vi "measure BT Frequency Separation Step1.vi"(8 "error in (no error)":errorcluster, 11 "SA Measurement in":refnum<class "SA Measurement.lvclass">) -> (0 "error out":errorcluster, 3 "SA Measurement out":refnum<class "SA Measurement.lvclass">)   [LabVIEW 2023, in "Spectrum Analyzer.lvlib" / "SA Measurement.lvclass"]
uses:
  SA Measurement.lvclass
  SA Measurement.lvclass/SA Measurement.ctl
  TYPE DEFINITION/Keysight 9020A/TYPE Measurement Preset.ctl
  Spectrum Analyzer.lvlib
  TYPE DEFINITION/TYPE RBW and VBW Select.ctl
  Interface_Spectrum/Interface_Spectrum.lvclass
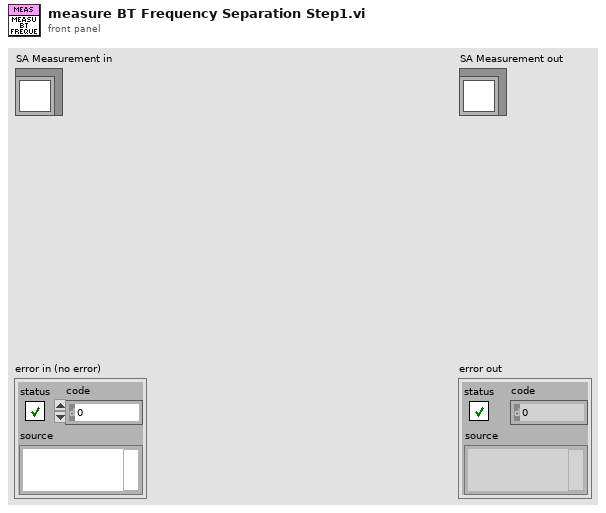
[diagram p1: front panel]
types:
  T1 = typedef "Spectrum Analyzer.lvlib/TYPE RBW and VBW Select.ctl" = enum16{"Res BW", "Video BW"}
  T2 = typedef "Spectrum Analyzer.lvlib/TYPE Measurement Preset.ctl" = enum16{"Sweep SA Mode", "Channel Power", "Occupied BW", "ACP", "Spurious Emission", "Spurious Emission Mask", "Burst Power (Transmit Power)"}
  T3 = typedef "Spectrum Analyzer.lvlib/TYPE Reference Level and Atten Param.ctl" = cluster{"Reference Level":dbl, "Atten":i32, "Atten Auto?":bool, "Reference Level Offset":dbl}
  T4 = typedef "Spectrum Analyzer.lvlib/TYPE Display Trace Mode Select.ctl" = enum16{"Clear Write", "Max Hold", "Min Hold", "Average", "View"}
  T5 = typedef "Spectrum Analyzer.lvlib/TYPE Detect Mode Select.ctl" = enum16{"Det Auto (Normal)", "Auto Peak", "Positive Peak", "Negative Peak", "Sample", "RMS", "Average", "Quasipeak", "CISPR Average", "RMS Average"}
  T6 = cluster{"Trace Mode":T4, "Detector Type":T5, "Detect Auto?":bool}[]
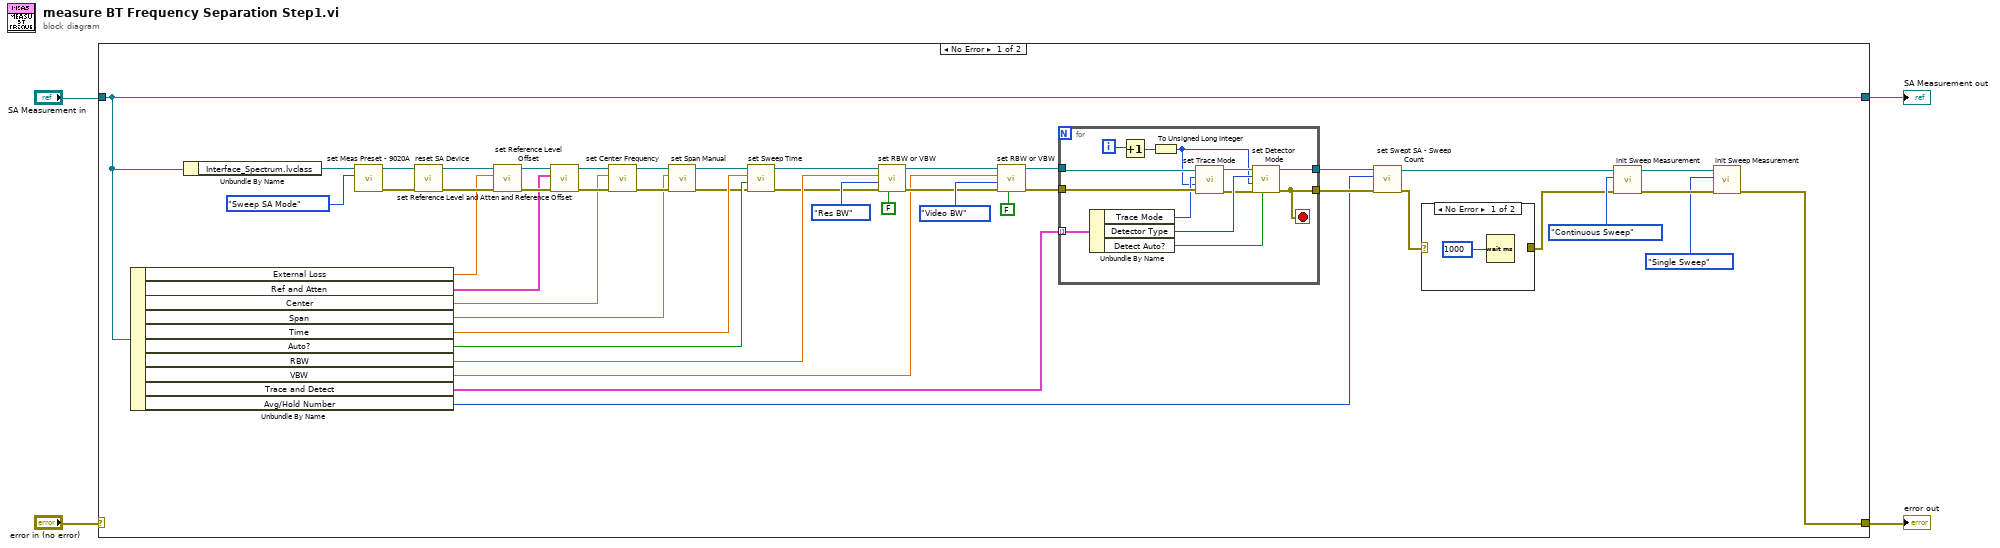
[diagram p0: block diagram]
diagram:
  n1 = case shown="No Error" "error in (no error)" {
    selector: "error in (no error)" -> [_ w66]
    tunnel: [w5 w66] -> w1
    tunnel: [w19 w65] -> w2
    tunnel: "SA Measurement in" -> [w19 w65]
    frame No Error {
      n2 = Unbundle By Name(w19) -> ("External Loss"=w41:dbl, "Ref and Atten"=w40:T3, "Center"=w16:dbl, "Span"=w13:dbl, "Time"=w25:dbl, "Auto?"=w24:bool, "RBW"=w33:dbl, "VBW"=w32:dbl, "Trace and Detect"=w29:T6, "Avg/Hold Number"=w26:u32)
      n3 = Unbundle By Name(w19) -> ("Interface_Spectrum.lvclass"=w49:refnum<class "Interface_Spectrum.lvclass">)
      n4 = call-dynamic "set Meas Preset - 9020A.vi"("Measurement Preset"=TYPE_Measurement_Preset."Sweep SA Mode", "Interface_Spectrum in"=w49) -> ("error out"=w46:errorcluster, "Interface_Spectrum out"=w47:refnum<class "Interface_Spectrum.lvclass">)  [unwired: 8 in]
      n5 = call-dynamic "reset SA Device.vi"("error in (no error)"=w46, "Interface_Spectrum in"=w47) -> ("error out"=w44:errorcluster, "Interface_Spectrum out"=w45:refnum<class "Interface_Spectrum.lvclass">)  [unwired: 8 in]
      n6 = call-dynamic "set Reference Level Offset.vi"("error in (no error)"=w44, "Reference Level Offset"=w41, "Interface_Spectrum in"=w45) -> ("error out"=w42:errorcluster, "Interface_Spectrum out"=w43:refnum<class "Interface_Spectrum.lvclass">)  [unwired: 7 in]
      n7 = call-dynamic "set Reference Level and Atten and Reference Offset.vi"("error in (no error)"=w42, "Reference Level, Atten, Reference Offset"=w40, "Interface_Spectrum in"=w43) -> ("error out"=w17:errorcluster, "Interface_Spectrum out"=w18:refnum<class "Interface_Spectrum.lvclass">)  [unwired: 7 in]
      n8 = call-dynamic "set Center Frequency.vi"("error in (no error)"=w17, "Center Frequency (Hz)"=w16, "Interface_Spectrum in"=w18) -> ("error out"=w14:errorcluster, "Interface_Spectrum out"=w15:refnum<class "Interface_Spectrum.lvclass">)  [unwired: 7 in]
      n9 = call-dynamic "set Span Manual.vi"("error in (no error)"=w14, "Span (Hz)"=w13, "Interface_Spectrum in"=w15) -> ("error out"=w11:errorcluster, "Interface_Spectrum out"=w12:refnum<class "Interface_Spectrum.lvclass">)  [unwired: 7 in]
      n10 = call-dynamic "set Sweep Time.vi"("error in (no error)"=w11, "Sweep Time Auto?"=w24, "Sweep Time(sec)"=w25, "Interface_Spectrum in"=w12) -> ("error out"=w22:errorcluster, "Interface_Spectrum out"=w23:refnum<class "Interface_Spectrum.lvclass">)  [unwired: 6 in]
      n11 = call-dynamic "set RBW or VBW.vi"("BW Auto?"=FALSE, "error in (no error)"=w22, "BW Type"=TYPE_RBW_and_VBW_Select."Res BW", "BW Value (Hz)"=w33, "Interface_Spectrum in"=w23) -> ("error out"=w34:errorcluster, "Interface_Spectrum out"=w35:refnum<class "Interface_Spectrum.lvclass">)  [unwired: 5 in]
      n12 = call-dynamic "set RBW or VBW.vi"("BW Auto?"=FALSE, "error in (no error)"=w34, "BW Type"=TYPE_RBW_and_VBW_Select."Video BW", "BW Value (Hz)"=w32, "Interface_Spectrum in"=w35) -> ("error out"=w30:errorcluster, "Interface_Spectrum out"=w31:refnum<class "Interface_Spectrum.lvclass">)  [unwired: 5 in]
      n13 = for {
        tunnel: w31 -> [w63]
        tunnel: w30 -> [w62]
        tunnel: w29 -> [w64] mode=indexing
        tunnel: [w52] -> w27
        tunnel: [w53] -> w28
        i -> [w61]
        stop <- w52 stop-if-true
        n14 = Unbundle By Name(w64) -> ("Trace Mode"=w59:T4, "Detector Type"=w57:T5, "Detect Auto?"=w54:bool)
        n15 = Increment(x=w61) -> (x+1=w60:i32)
        n16 = To Unsigned Long Integer(number=w60) -> (unsigned 32bit integer=w55:u32)
        n17 = call-dynamic "set Trace Mode.vi"("error in (no error)"=w62, "Trace Index"=w55, "Trace Mode"=w59, "Interface_Spectrum in"=w63) -> ("error out"=w56:errorcluster, "Interface_Spectrum out"=w58:refnum<class "Interface_Spectrum.lvclass">)  [unwired: 6 in]
        n18 = call-dynamic "set Detector Mode.vi"("Detect Auto?"=w54, "error in (no error)"=w56, "Trace Index"=w55, "Detector Type"=w57, "Interface_Spectrum in"=w58) -> ("error out"=w52:errorcluster, "Interface_Spectrum out"=w53:refnum<class "Interface_Spectrum.lvclass">)  [unwired: 5 in]
      }
      n19 = call-dynamic "set Swept SA - Sweep Count.vi"("error in (no error)"=w27, "Sweep Count"=w26, "Interface_Spectrum in"=w28) -> ("error out"=w10:errorcluster, "Interface_Spectrum out"=w21:refnum<class "Interface_Spectrum.lvclass">)  [unwired: 7 in]
      n20 = case shown="No Error" w10 {
        selector: w10 -> [_ w51]
        tunnel: [_ w51] -> w9
        frame No Error {
          n21 = Wait (ms)(milliseconds to wait=u32 1000) -> ()  [unwired: 1 out]
        }
        frame Error {
        }
      }
      n22 = call-dynamic "init Sweep Measurement.vi"("error in (no error)"=w9, "Sweep Measurement Mode"=enum16{"Single Sweep", "Continuous Sweep"}."Continuous Sweep", "Interface_Spectrum in"=w21) -> ("error out"=w7:errorcluster, "Interface_Spectrum out"=w8:refnum<class "Interface_Spectrum.lvclass">)  [unwired: 7 in]
      n23 = call-dynamic "init Sweep Measurement.vi"("error in (no error)"=w7, "Sweep Measurement Mode"=enum16{"Single Sweep", "Continuous Sweep"}."Single Sweep", "Interface_Spectrum in"=w8) -> ("error out"=w5:errorcluster)  [unwired: 7 in, 1 out]
    }
    frame Error {
    }
  }
  "error out" <- w1
  "SA Measurement out" <- w2
